vi "ThroughBore Calibration.vi"(11 "(N-N-C-P) Swerve Motors":T1 {"Steer Scaling" format="%.2f"; "Drive Scaling" format="%.2f"; "Pod Locations (ft)"."Right Back Position" format="%.2f"; "Pod Locations (ft)"."Right Front Position" format="%.2f"; "Pod Locations (ft)"."Left Back Position" format="%.2f"; "Pod Locations (ft)"."Left Front Position" format="%.2f"}) -> (0 "error out":errorcluster, 3 "Steering Angles":cluster{"LF":dbl, "LB":dbl, "RF":dbl, "RB":dbl})   [LabVIEW 2027]
uses:
  Type Definitions/Hardware/Swerve Drives/(NEO-NEO-ThroughBore-Pigeon2) Swerve.ctl
  <vilib>/REV Custom Controls/REVSparkRefnum.ctl
  Type Definitions/Data/Pod Positions.ctl
  <vilib>/Analysis/coordinate.llb/Angle Units.ctl
  <vilib>/Analysis/coordinate.llb/Wrap Angle (scalar).vi
  <vilib>/Analysis/NI_AAL_Angle.lvlib
  <resource>/objmgr/REVSpark.rc
  <vilib>/REVLibDriver/REVLibDriver.lvlib
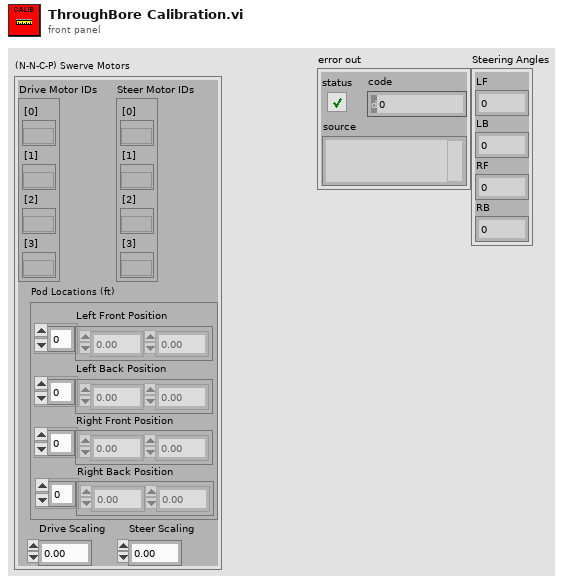
[diagram p1: front panel]
types:
  T1 = typedef "(NEO-NEO-ThroughBore-Pigeon2) Swerve.ctl" = cluster{"Drive Motor IDs":cluster{"[0]":T2, "[1]":T2, "[2]":T2, "[3]":T2}, "Steer Motor IDs":cluster{"[0]":T2, "[1]":T2, "[2]":T2, "[3]":T2}, "Pod Locations (ft)":T3, "Drive Scaling":dbl, "Steer Scaling":dbl}
  T2 = typedef "REVLibDriver.lvlib/REVSparkRefnum.ctl" = refnum<k20>
  T3 = typedef "Pod Positions.ctl" = cluster{"Left Front Position":dbl[], "Left Back Position":dbl[], "Right Front Position":dbl[], "Right Back Position":dbl[]}
  T4 = typedef "NI_AAL_Angle.lvlib/Angle Units.ctl" = i32
  T5 = cluster{"[0]":dbl, "[1]":dbl, "[2]":dbl, "[3]":dbl}
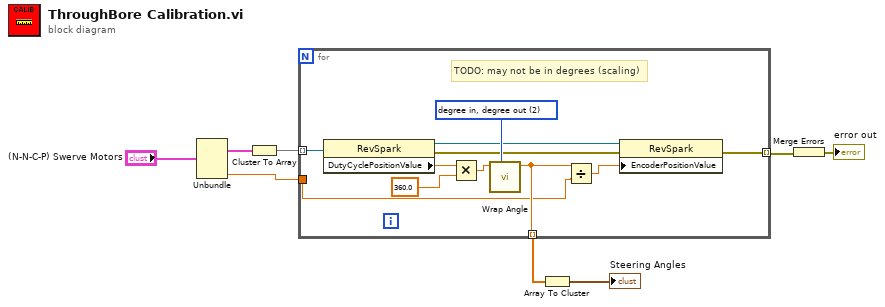
[diagram p0: block diagram]
diagram:
  n1 = Unbundle("(N-N-C-P) Swerve Motors") -> ("Steer Motor IDs"=w7:cluster{"[0]":T2, "[1]":T2, "[2]":T2, "[3]":T2}, "Steer Scaling"=w1:dbl)  [unwired: 3 out]
  n2 = Cluster To Array(cluster=w7) -> (array=w6:T2[])
  n3 = for {
    tunnel: w6 -> [w18] mode=indexing
    tunnel: [w16] -> w5 mode=indexing
    tunnel: [w12] -> w3 mode=indexing
    tunnel: w1 -> [w11]
    w19 = T4 2 items=["radian in, radian out", "radian in, degree out", "degree in, degree out", "degree in, radian out"] ("angle units")
    # "TODO: may not be in degrees (scaling)"
    n4 = property class="RevSpark"(reference=w18) -> (reference out=w17:T2, error out=w15:errorcluster, "DutyCyclePositionValue"=w13:sgl)  [unwired: 1 in]
    n5 = Multiply(x=w13, y=sgl 360.0) -> (x*y=w14:sgl)
    n6 = call-poly <vilib>:"Wrap Angle.vi"("angle units"=w19, "angle in"=w14) -> ("angle out"=w12:dbl)  [unwired: 8 in, 1 out]
    n7 = Divide(x=w12, y=w11) -> (x/y=w10:dbl)
    n8 = property class="RevSpark"(reference=w17, error in=w15, "EncoderPositionValue"=w10) -> (error out=w16:errorcluster)  [unwired: 1 out]
  }
  n9 = Array To Cluster(array=w3) -> (cluster=→"Steering Angles":T5)
  n10 = Merge Errors(w5) -> (→"error out":errorcluster)
